vi "OpenG Array filter -Regexp Invert  Scalar Template.vi"() -> ()   [LabVIEW 2012]
panel:
  out "filtered item indices":i32[](array[numeric])
  out "filtered array":string[](array[string])
  in  "items to filter":string
  in  "Array Input":string[](array[string])
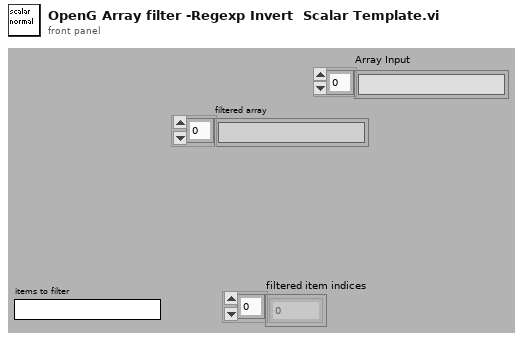
[diagram p1: front panel]
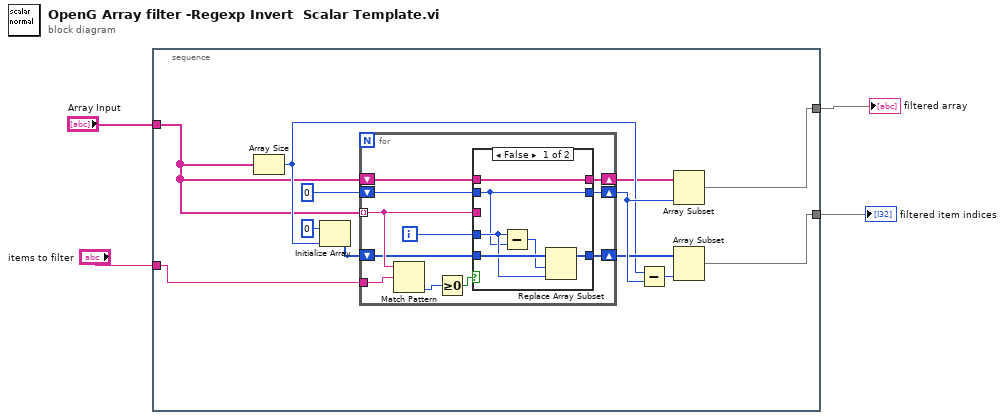
[diagram p0: block diagram]
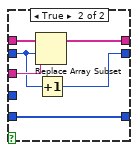
[diagram p2: hidden frame]
diagram:
  n1 = stacked-sequence {
    tunnel: "items to filter" -> [w8]
    tunnel: [w6] -> w3
    tunnel: "Array Input" -> [w7]
    tunnel: [w5] -> w1
    frame #0 {
      n2 = Array Size(array=w7) -> (size(s)=w13:i32)
      n3 = Initialize Array(0 ("Numeric"), w13) -> (w12:i32[])
      n4 = for {
        tunnel: w7 -> [w25] mode=indexing
        shift-right: [w26] -> w10
        shift-left: w7 -> [w27]
        shift-right: [w23] -> w15
        shift-left: 0 -> [w24]
        shift-right: [w21] -> w14
        shift-left: w12 -> [w22]
        tunnel: w8 -> [w20]
        i -> [w19]
        n5 = Match Pattern(string=w25, regular expression=w20) -> (offset past match=w18:i32)  [unwired: 4 out]
        n6 = Greater Or Equal To 0?(x=w18) -> (x >= 0?=w17:bool)
        n7 = case shown="False" w17 {
          tunnel: w27 -> [w33 w39]
          tunnel: [w33 w38] -> w26
          tunnel: w25 -> [_ w37]
          tunnel: w24 -> [w29 w35]
          tunnel: [w29 w36] -> w23
          tunnel: w22 -> [w32 w34]
          tunnel: [w31 w34] -> w21
          tunnel: w19 -> [w30 _]
          frame False {
            n8 = Subtract(x=w30, y=w29) -> (x-y=w28:i32)
            n9 = Replace Array Subset(array=w32, new element=w30, index=w28) -> (w31:i32[])
          }
          frame True {
            n10 = Replace Array Subset(array=w39, new element=w37, index=w35) -> (w38:string[])
            n11 = Increment(x=w35) -> (x+1=w36:i32)
          }
        }
      }
      n12 = Subtract(x=w13, y=w15) -> (x-y=w16:i32)
      n13 = Array Subset(array=w10, length=w15) -> (w5:string[])  [unwired: 1 in]
      n14 = Array Subset(array=w14, length=w16) -> (w6:i32[])  [unwired: 1 in]
    }
  }
  "filtered array" <- w1
  "filtered item indices" <- w3
